vi "optical_grab2.vi"() -> ()   [LabVIEW 2025]
uses:
  <vilib>/vision/driver/NI_Vision_Acquisition_Software.lvlib
panel:
  out "Image Preview":T1(plugin-control)
  out "error out":errorcluster
  out "FPS":u32
  in  "Output Folder":path
  in  "Stop":bool
  in  "Camera Name":refnum<k21> caption="IMAQdx Session"
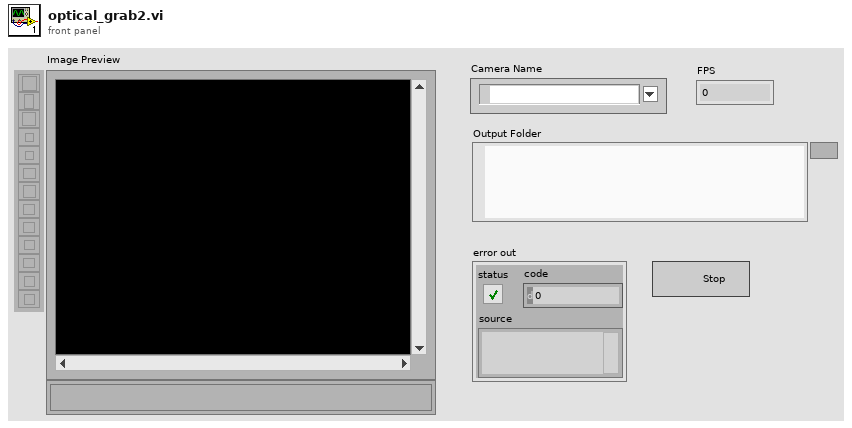
[diagram p1: front panel]
types:
  T1 = typedef "IMAQ Image.ctl" = refnum<image>
  T2 = typedef "Image Type" = u32
  T3 = typedef "IMAQdx.ctl" = refnum<k21>
  T4 = enum16{"big-endian, network order", "native, host order", "little-endian"}
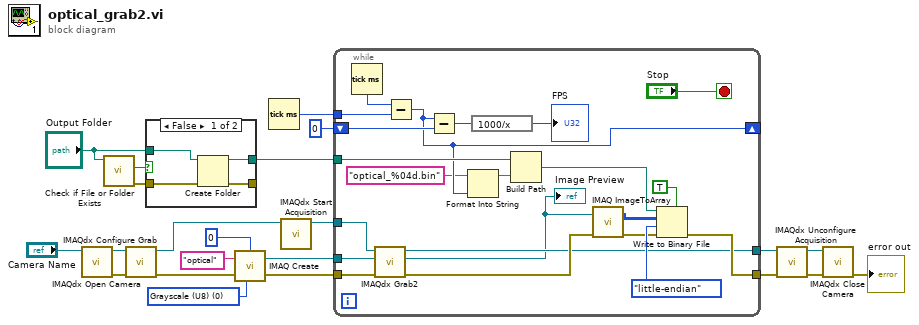
[diagram p0: block diagram]
diagram:
  w13 = T2 0 items=["Grayscale (U8)", "Grayscale (I16)", "Grayscale (SGL)", "Complex (CSG)", "RGB (U32)", "HSL (U32)", "RGB (U64)", "Grayscale (U16)"] ("Image Type")
  n1 = call <vilib>:"IMAQdx Open Camera.vi"("Session In"="Camera Name") -> ("error out"=w6:errorcluster, "Session Out"=w8:T3)  [unwired: 9 in]
  n2 = call <vilib>:"Check if File or Folder Exists.vi"("path"="Output Folder") -> ("error out"=w20:errorcluster, "file or folder exists?"=w22:bool)  [unwired: 8 in, 1 out]
  n3 = call <vilib>:"IMAQdx Configure Grab.vi"("error in"=w6, "Session In"=w8) -> ("error out"=w5:errorcluster, "Session Out"=w7:T3)  [unwired: 8 in]
  n4 = case shown="False" w22 {
    tunnel: "Output Folder" -> [w26 w28]
    tunnel: [w25 w28] -> w19
    tunnel: w20 -> [w24 w27]
    tunnel: [w23 w27] -> _
    frame False {
      n5 = Create Folder(path (use dialog)=w26, error in=w24) -> (created path=w25:path, error out=w23:errorcluster)  [unwired: 1 in, 1 out]
    }
    frame True {
    }
  }
  n6 = call "IMAQ Create"("Border Size"=0, "Image Name"="optical", "Image Type"=w13, "error in (no error)"=w5) -> ("New Image"=w10:T1, "error out"=w9:errorcluster)  [unwired: 1 in]
  n7 = Tick Count (ms)() -> (millisecond timer value=w18:u32)
  n8 = call <vilib>:"IMAQdx Start Acquisition.vi"("Session In"=w7) -> ("Session Out"=w11:T3)  [unwired: 9 in, 1 out]
  n9 = while {
    tunnel: w19 -> [w50]
    tunnel: w18 -> [w48]
    shift-right: [w46] -> _
    shift-left: u32 0 -> [w47]
    tunnel: w11 -> [w42]
    tunnel: w10 -> [w41]
    tunnel: w9 -> [w40]
    tunnel: [w31] -> w4
    tunnel: [w37] -> w1
    stop <- "Stop" stop-if-true
    n10 = Tick Count (ms)() -> (millisecond timer value=w49:u32)
    n11 = call <vilib>:"IMAQdx Grab2.vi"("error in"=w40, "Image In"=w41, "Session In"=w42) -> ("error out"=w39:errorcluster, "Image Out"=w30:T1, "Session Out"=w31:T3)  [unwired: 5 in, 1 out]
    "Image Preview" <- w30
    n12 = Subtract(x=w49, y=w48) -> (x-y=w46:u32)
    n13 = Subtract(x=w46, y=w47) -> (x-y=w33:u32)
    n14 = Format Into String(format string="optical_%04d.bin", w46) -> (resulting string=w45:string)  [unwired: 2 in, 1 out]
    n15 = expression code="1000/x"(w33) -> (→"FPS":u32)
    n16 = Build Path(base path=w50, name or relative path=w45) -> (appended path=w38:path)
    n17 = call "IMAQ ImageToArray"("error in (no error)"=w39, "Image"=w30) -> ("error out"=w34:errorcluster, "Image Pixels (U8)"=w29:u8[][])  [unwired: 2 in, 3 out]
    n18 = Write to Binary File(file (use dialog)=w38, data=w29, error in=w34, 5:TRUE, 9:T4."little-endian" ("byte order (0:big-endian, network order)")) -> (error out=w37:errorcluster)  [unwired: 1 in, 2 out]
  }
  n19 = call <vilib>:"IMAQdx Unconfigure Acquisition.vi"("error in"=w1, "Session In"=w4) -> ("error out"=w2:errorcluster, "Session Out"=w3:T3)  [unwired: 8 in]
  n20 = call <vilib>:"IMAQdx Close Camera.vi"("error in"=w2, "Session In"=w3) -> ("error out"=→"error out":errorcluster)  [unwired: 9 in]
